vi "Runner Tests.vi"(8 "error in (no error)":errorcluster) -> (0 "error out":errorcluster)   [LabVIEW 2020]
uses:
  classes/Test Runner/Test Runner.lvclass
  test-all-asserts/Test Runner.AllAsserts.lvclass
  C:/projects/caraya/src/classes/Test Runner/Test Runner.lvclass
  classes/Test Runner.Project/Test Runner.Project.lvclass
  classes/Test Runner.Library/Test Runner.Library.lvclass
  UnitTest For Runner/Unit Tests for Runner.lvclass
  classes/Test Runner.Folder/Test Runner.Folder.lvclass
  classes/Test Runner.Collection/Test Runner.Collection.lvclass
  classes/Test/Test.lvclass
  classes/Assert/Assert.lvclass
  Caraya.lvlib
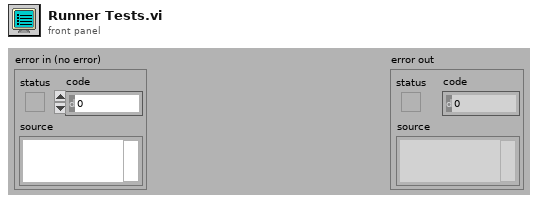
[diagram p1: front panel]
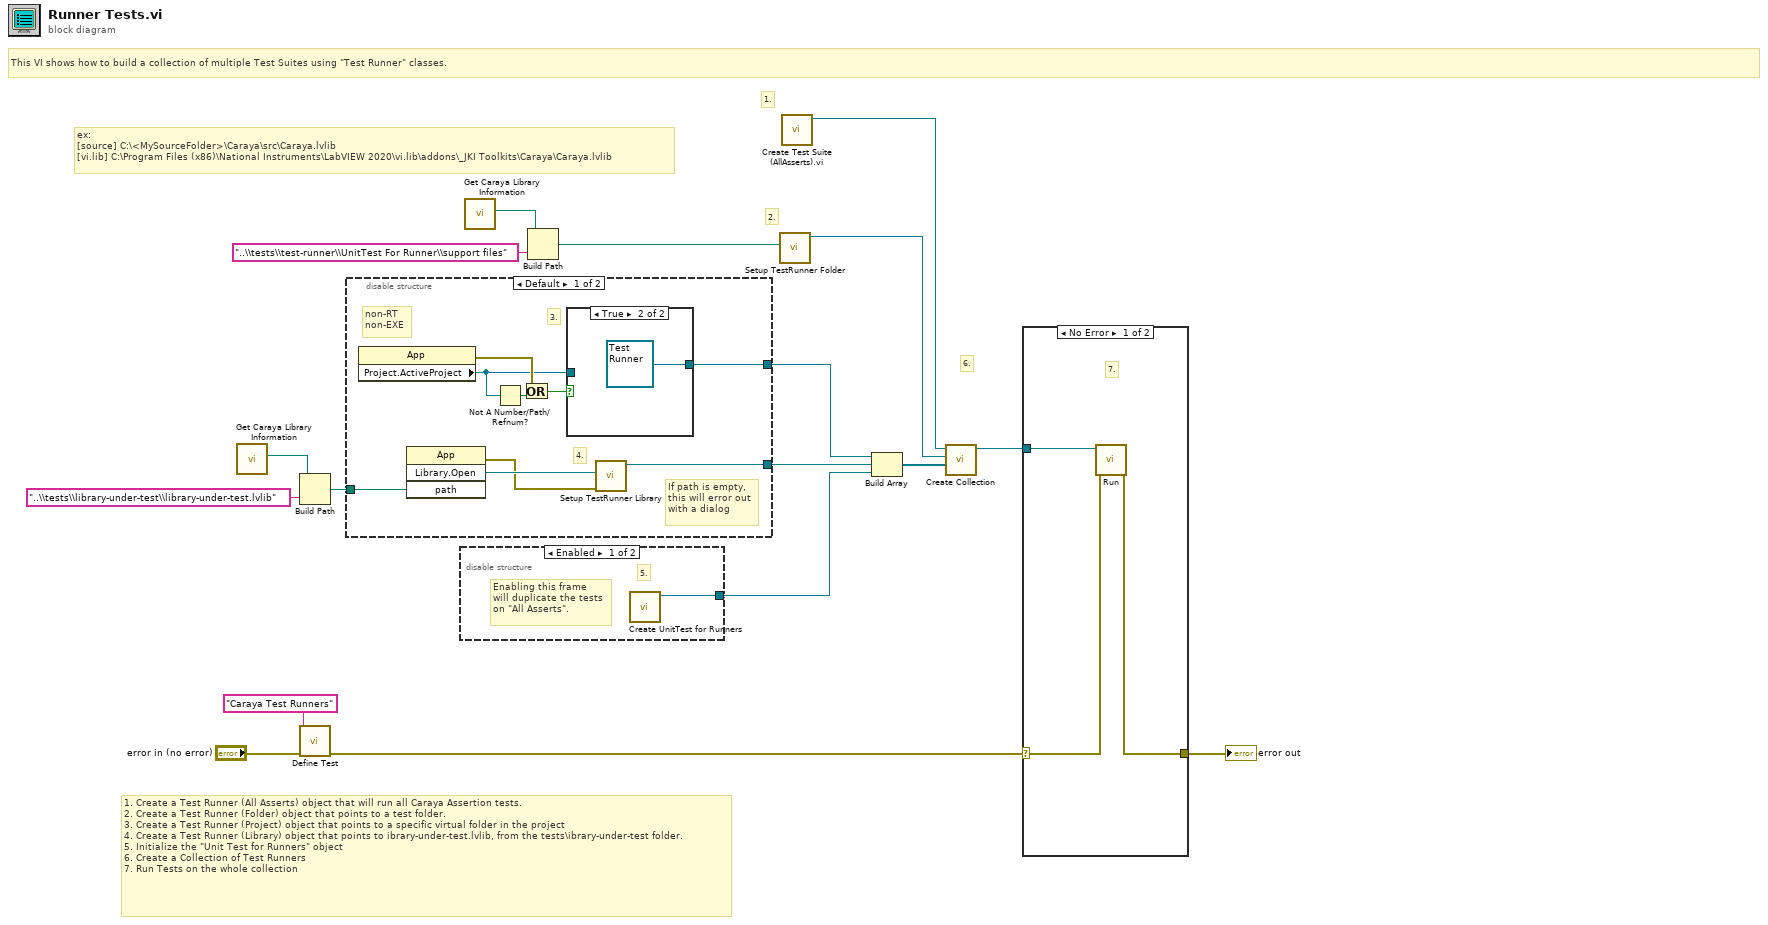
[diagram p0: block diagram]
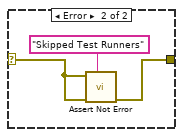
[diagram p2: hidden frame]
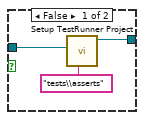
[diagram p3: hidden frame]
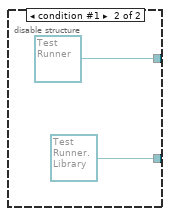
[diagram p4: hidden frame]
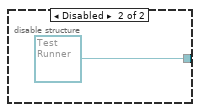
[diagram p5: hidden frame]
diagram:
  # "ex: \n[source] C:\\<MySourceFolder>\\Caraya\\src\\Caraya.lvlib\n[vi.lib] C:\\Program Files (x86)\\National Instruments\\LabVIEW 2020\\vi.lib\\addons\\_JKI Toolkits\\Caraya\\Caraya.lvlib"
  # "This VI shows how to build a collection of multiple Test Suites using \"Test Runner\" classes."
  # "1."
  # "1. Create a Test Runner (All Asserts) object that will run all Caraya Assertion tests.\n2. Create a Test Runner (Folder) object that points to a test folder.\n3. Create a Test Runner (Project) object that points to a specific virtual folder in the project\n4. Create a Test Runner (Library) object that points to ibrary-under-test.lvlib, from the tests\\ibrary-under-test folder.\n5. Initialize the \"Unit Test for Runners\" object\n6. Create a Collection of Test Runners\n7. Run Tests on the whole collection"
  # "6."
  # "2."
  n1 = call "Get Caraya Library Information.vi"() -> ("Caraya Library Path"=w6:path)  [unwired: 9 in, 2 out]
  n2 = Build Path(base path=w6, name or relative path="..\\tests\\library-under-test\\library-under-test.lvlib") -> (appended path=w4:path)
  n3 = call "Define Test.vi"("error in (no error)"="error in (no error)", "Label (VI Title)"="Caraya Test Runners") -> ("error out"=w7:errorcluster)  [unwired: 8 in, 1 out]
  n4 = disable-structure shown="Default" {
    disable-tunnel: [w22 refnum<class "Test Runner.lvclass"> refnum ("Test Runner 2")] -> w14
    disable-tunnel: w4 -> [w21 _]
    disable-tunnel: [w19 refnum<class "Test Runner.Library.lvclass"> refnum ("Test Runner.Library out")] -> w11
    frame condition #0 (active) {
      # "If path is empty, \nthis will error out\nwith a dialog"
      # "4."
      # "non-RT\nnon-EXE"
      # "3."
      n5 = property on="Property Node" class="App"() -> (error out=w25:errorcluster, "Project.ActiveProject"=w24:refnum<vi>)  [unwired: 2 in, 1 out]
      n6 = invoke class="App" method="Library.Open"("path"=w21) -> (error out=w18:errorcluster, "Open Library"=w20:refnum<vi>)  [unwired: 3 in, 2 out]
      n7 = Not A Number/Path/Refnum?(number/path/refnum=w24) -> (NaN/Path/Refnum?=w26:bool)
      n8 = Or(x=w25, y=w26) -> (x .or. y?=w23:bool)
      n9 = case shown="True" w23 {
        tunnel: [w29 refnum<class "Test Runner.lvclass"> refnum ("Test Runner 2")] -> w22
        tunnel: w24 -> [w27 _]
        frame False {
          n10 = call "Setup TestRunner Project.vi"("Virtual Folder (empty: \"My Computer\")"="tests\\asserts" ("Virtual Folder (empty: \"My Computer\")"), "Project Refnum"=w27) -> ("Test Runner.Project out"=w29:refnum<class "Test Runner.Project.lvclass">)  [unwired: 8 in, 1 out]
        }
        frame True {
        }
      }
      n11 = call "Setup TestRunner Library.vi"("error in (no error)"=w18, "Library Refnum"=w20) -> ("Test Runner.Library out"=w19:refnum<class "Test Runner.Library.lvclass">)  [unwired: 8 in, 1 out]
    }
    frame condition #1 {
    }
  }
  n12 = disable-structure shown="Enabled" {
    disable-tunnel: [w33 refnum<class "Test Runner.lvclass"> refnum ("Test Runner 2")] -> w16
    frame Enabled {
      # "Enabling this frame\nwill duplicate the tests\non \"All Asserts\"."
      # "5."
      n13 = call "Create UnitTest for Runners.vi"() -> ("Unit Tests for Runner out"=w33:refnum<class "Unit Tests for Runner.lvclass">)  [unwired: 10 in, 1 out]
    }
    frame Disabled {
    }
  }
  n14 = call "Get Caraya Library Information.vi"() -> ("Caraya Library Path"=w2:path)  [unwired: 9 in, 2 out]
  n15 = Build Path(base path=w2, name or relative path="..\\tests\\test-runner\\UnitTest For Runner\\support files") -> (appended path=w1:path)
  n16 = call "Setup TestRunner Folder.vi"("Directory to search"=w1) -> ("Test Runner.Folder out"=w13:refnum<class "Test Runner.Folder.lvclass">)  [unwired: 9 in, 1 out]
  n17 = call "Create Test Suite (AllAsserts).vi.vi"() -> ("Test Runner.AllAsserts in"=w12:refnum<class "Test Runner.AllAsserts.lvclass">)  [unwired: 10 in, 1 out]
  n18 = Build Array(w14, w11, w16) -> (w15:refnum<class "Test Runner.lvclass">[])
  n19 = call "Create Collection.vi"("Test Runners"=w15, "Test Runner 2"=w13, "Test Runner 1"=w12) -> ("Test Runner.Collection out"=w17:refnum<class "Test Runner.Collection.lvclass">)  [unwired: 7 in, 1 out]
  n20 = case shown="No Error" w7 {
    selector: w7 -> [w35 w39]
    tunnel: w17 -> [w37 _]
    tunnel: [w36 w38] -> w8
    frame No Error {
      # "7."
      n21 = call "Run.vi"("error in (no error)"=w35, "Test Runner in"=w37) -> ("error out"=w36:errorcluster)  [unwired: 7 in, 2 out]
    }
    frame Error {
      n22 = call "Assert Not Error.vi"("Label"="Skipped Test Runners" ("Label (VI Title)"), "error in (no error)"=w39, "Not Error?"=w39) -> ("error out"=w38:errorcluster)  [unwired: 7 in, 1 out]
    }
  }
  "error out" <- w8
